vi "Test Verbose Report.vi"() -> ()   [LabVIEW 2020]
uses:
  classes/Test Result/Node Results.ctl
  classes/Test Result/Test Node.ctl
  classes/Test Result/Test Registration Data.ctl
  classes/Test Result/Assert Event Data.ctl
  classes/Test Suite/Test Suite.lvclass
  classes/Test Result/Test Result.lvclass
panel:
  out "Test Results":T1[](array[typedef])
  out "error out":errorcluster
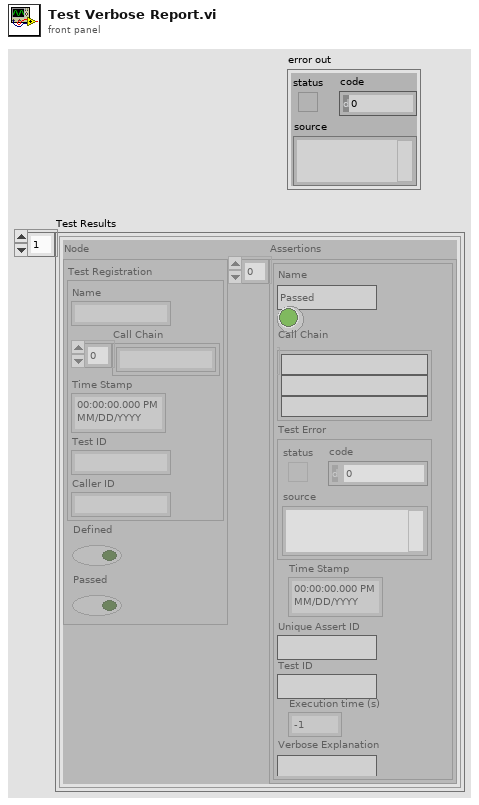
[diagram p1: front panel]
types:
  T1 = typedef "Caraya.lvlib/Test Result.lvclass/Node Results.ctl" = cluster{"Node":T2, "Assertions":T4[]}
  T2 = typedef "Caraya.lvlib/Test Result.lvclass/Test Node.ctl" = cluster{"Test Registration":T3, "Defined":bool, "Passed":bool}
  T3 = typedef "Caraya.lvlib/Test Result.lvclass/Test Registration Data.ctl" = cluster{"Name":string, "Call Chain":string[], "Time Stamp":timestamp, "Test ID":string, "Caller ID":string}
  T4 = typedef "Caraya.lvlib/Test Result.lvclass/Assert Event Data.ctl" = cluster{"Name":string, "Passed":bool, "Call Chain":string[], "Test Error":errorcluster, "Time Stamp":timestamp, "Unique Assert ID":string, "Test ID":string, "Execution time (s)":dbl, "Verbose Explanation":string}
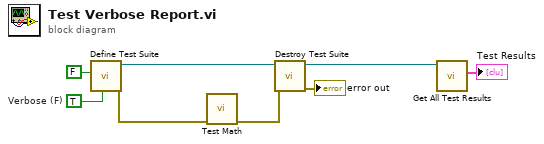
[diagram p0: block diagram]
diagram:
  w8 = TRUE  # Verbose (F)
  n1 = call "Define Test Suite.vi"("Verbose (F)"=w8, "Interactive"=FALSE) -> ("error out"=w6:errorcluster, "Test Suite"=w7:refnum<class "Test Suite.lvclass">)  [unwired: 7 in, 1 out]
  n2 = call "Test Math.vi"("error in (no error)"=w6) -> ("error out"=w5:errorcluster)  [unwired: 10 in]
  n3 = call-dynamic "Destroy Test Suite.vi"("error in (no error)"=w5, "Test Suite in"=w7) -> ("error out"=→"error out":errorcluster, "Test Suite Results"=w2:refnum<class "Test Result.lvclass">)  [unwired: 8 in]
  n4 = call "Get All Test Results.vi"("Test Result in"=w2) -> ("Test Results"=→"Test Results":T1[])  [unwired: 8 in, 2 out]
